vi "main_test_lab2_3.vi"() -> ()   [LabVIEW 2025]
uses:
  <vilib>/rvi/DesktopExecutionNode/DesktopExecutionNode.xnode
  <vilib>/rvi/DesktopExecutionNode/Execution/niFpgaDEN_Execute.vi
panel:
  out "Waveform Acc Now":T1(graph)
  out "Waveform Acc Max":T2(graph)
  in  "Shake left":bool
  in  "Shake forward":bool
  out "Mean X":fxp<+/-,64,33>
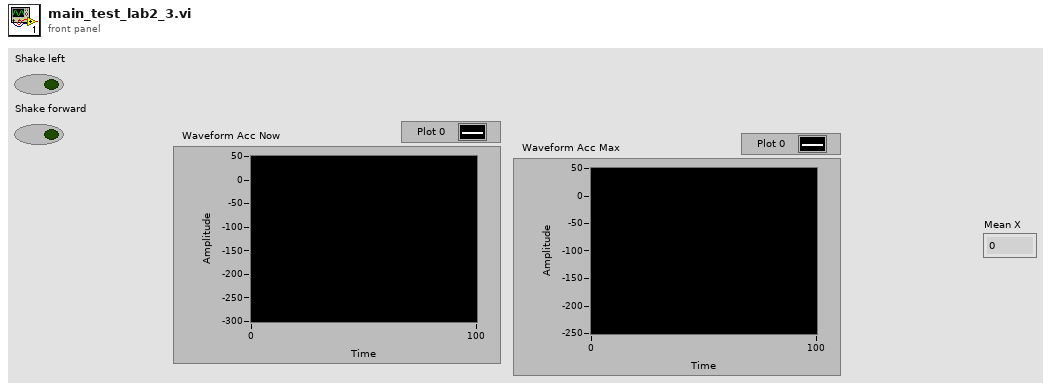
[diagram p1: front panel]
types:
  T1 = cluster{"AccelerationX Now":i16, "AccelerationY Now":i16, "AccelerationZ Now":i16}
  T2 = cluster{"AccelerationX Max":i16, "AccelerationY Max":i16, "AccelerationZ Max":i16}
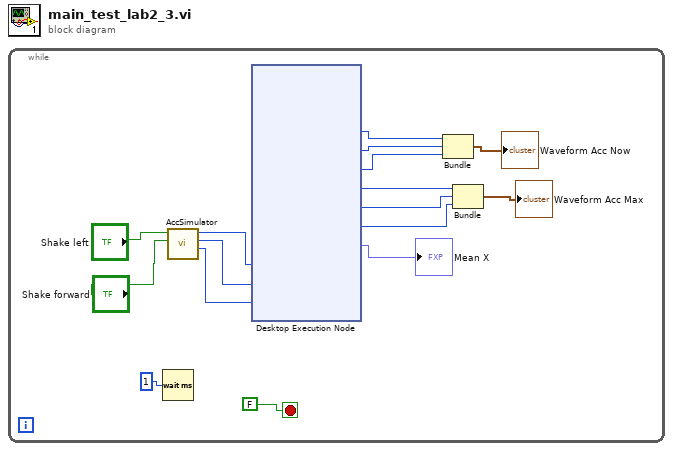
[diagram p0: block diagram]
diagram:
  n1 = while {
    stop <- FALSE stop-if-true
    n2 = Wait (ms)(milliseconds to wait=u32 1) -> ()  [unwired: 1 out]
    n3 = call "AccSimulator.vi"("Shake forward"="Shake forward", "Shake left"="Shake left") -> ("Acc Y"=w1:i16, "Acc X"=w2:i16, "Acc Z"=w3:i16)  [unwired: 7 in]
    n4 = xnode "Desktop Execution Node"("AccelerationZ"=w3, "AccelerationX"=w2, "AccelerationY"=w1) -> ("AccelerationX Now"=w12:i16, "AccelerationY Now"=w11:i16, "AccelerationZ Now"=w10:i16, "AccelerationX Max"=w9:i16, "AccelerationY Max"=w8:i16, "AccelerationZ Max"=w7:i16, "Mean X"=→"Mean X":fxp<+/-,64,33>)  [unwired: 1 in, 1 out]
    n5 = Bundle("AccelerationX Now"=w12, "AccelerationY Now"=w11, "AccelerationZ Now"=w10) -> (→"Waveform Acc Now":T1)  [unwired: 1 in]
    n6 = Bundle("AccelerationX Max"=w9, "AccelerationY Max"=w8, "AccelerationZ Max"=w7) -> (→"Waveform Acc Max":T2)  [unwired: 1 in]
  }
